vi "Process Acknowledgement.vi"(8 "error in (no error)":errorcluster, 10 "Incoming Packet":refnum<class "ControlPacket.lvclass">, 11 "Session in":refnum<class "Session.lvclass">) -> (0 "error out":errorcluster, 3 "Session out":refnum<class "Session.lvclass">)   [LabVIEW 2013, in "MQTT Base.lvlib" / "Session.lvclass"]
uses:
  Session.lvclass
  <vilib>/LabVIEW Open Source Project/MQTT Control Packets/Control Packets/ControlPacket/ControlPacket.lvclass
  Base Class/Response -- cluster.ctl
  Session.lvclass/Session.ctl
  Base Class/MQTT_Base.lvclass
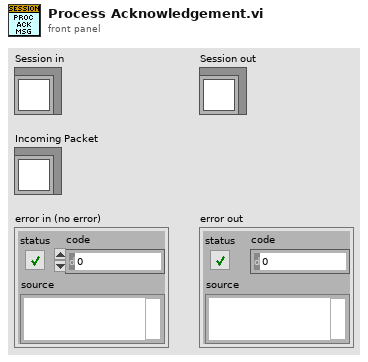
[diagram p1: front panel]
types:
  T1 = typedef "MQTT Base.lvlib/MQTT_Base.lvclass/Response -- cluster.ctl" = cluster{"Packet":refnum<class "ControlPacket.lvclass">, "Protocol Error":errorcluster, "disconnect session":bool, "[ACK]":refnum<notifier>[]}
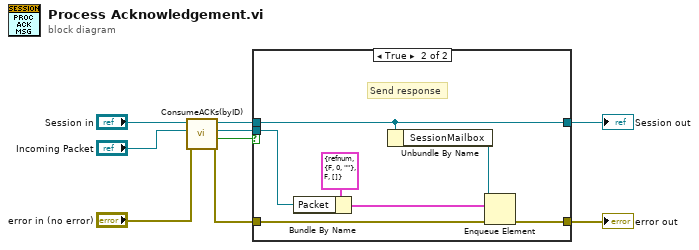
[diagram p0: block diagram]
diagram:
  n1 = call "ConsumeACKs(byID).vi"("error in (no error)"="error in (no error)", "ControlPacket in"="Incoming Packet", "Session in"="Session in") -> ("error out"=w1:errorcluster, "response prepared?"=w5:bool, "ControlPacket response"=w6:refnum<class "ControlPacket.lvclass">, "Session out"=w7:refnum<class "Session.lvclass">)  [unwired: 5 in]
  n2 = case shown="True" w5 {
    tunnel: w7 -> [w11 w13]
    tunnel: [w10 w16] -> w2
    tunnel: [w11 w13] -> w8
    tunnel: w6 -> [_ w15]
    tunnel: w1 -> [w10 w14]
    frame False {
    }
    frame True {
      # "Send response"
      n3 = Bundle By Name(cluster=T1 {"Packet"=refnum, "Protocol Error"={"status"=FALSE, "code"=0, "source"=""}, "disconnect session"=FALSE, "[ACK]"=[]} ("element"), "Packet"=w15) -> (w17:T1)
      n4 = Unbundle By Name(w13) -> ("SessionMailbox"=w12:refnum<queue>)
      n5 = Enqueue Element(queue=w12, element=w17, error in (no error)=w14) -> (error out=w16:errorcluster)  [unwired: 1 in, 2 out]
    }
  }
  "Session out" <- w8
  "error out" <- w2
